vi "Lab 4.vi"() -> ()   [LabVIEW 2025]
uses:
  Lab 4/Control ENUM.ctl
  Lab 3/Control og.ctl
  Lab 3/Control Runners.ctl
  Lab 3/Control Raw.ctl
  <vilib>/Analysis/baseanly.llb/Mean (DBL).vi
  <vilib>/Analysis/NI_AALBase.lvlib
panel:
  in  "File Path":path
  out "HEART RATE ZONES":string[][](array[string])
  out "BPM":cluster{"Time":timestamp[], "Bpm":i32[]}(graph)
  out "XY Graph":T1(graph)
  in  "Stop":bool
  in  "Save":bool
  in  "New":bool
  out "error out":errorcluster
  in  "error in":errorcluster
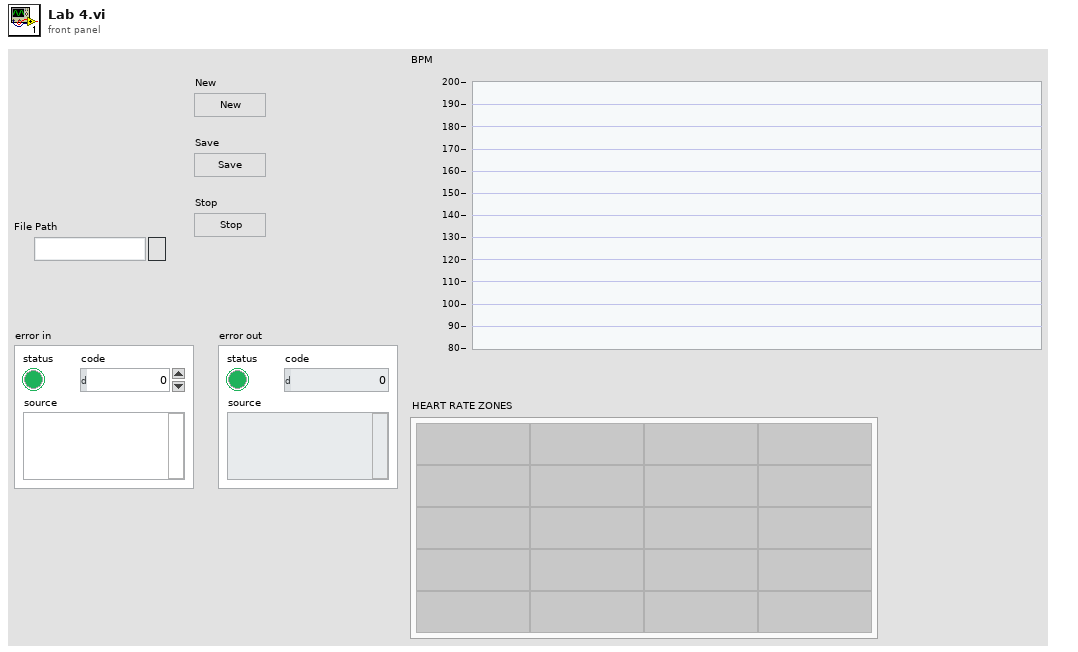
[diagram p1: front panel]
types:
  T1 = cluster{"Total Time in Zone":dbl[], "Heart Rate Zone No":dbl[]}
  T2 = typedef "Control og.ctl" = cluster{"Runner's Data":T3, "HR Max":i32, "Raw Data":T4, "% HR MAX ":dbl[], "HR Zones":string[][], "Heart Rate Zone No":dbl[], "Total Time in Zone":dbl[]}
  T3 = typedef "Control Runners.ctl" = cluster{"Name":string, "Age":i32}
  T4 = typedef "Control Raw.ctl" = cluster{"Time":timestamp[], "Bpm":i32[]}
  T5 = typedef "Control ENUM.ctl" = enum16{"Application Error", "Init", "Idle", "Analyse New Training", "Save", "Error Handling", "Stop"}
  T6 = enum16{"open", "replace", "create", "open or create", "replace or create", "replace or create with confirmation"}
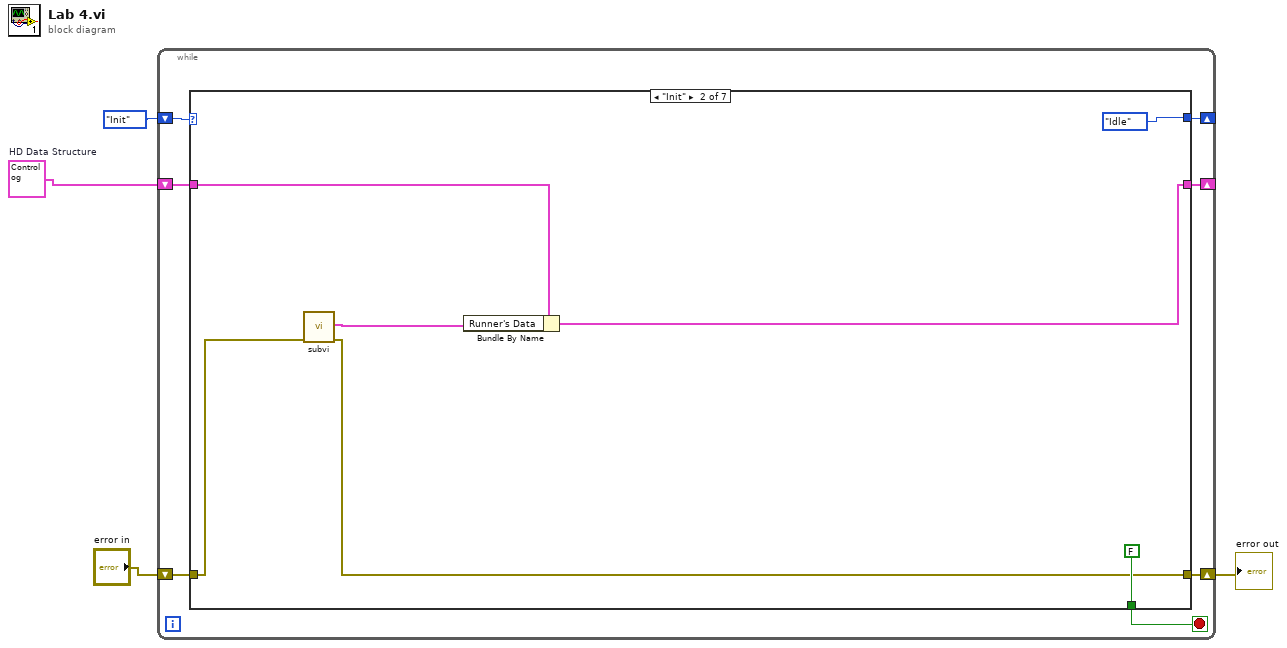
[diagram p0: block diagram]
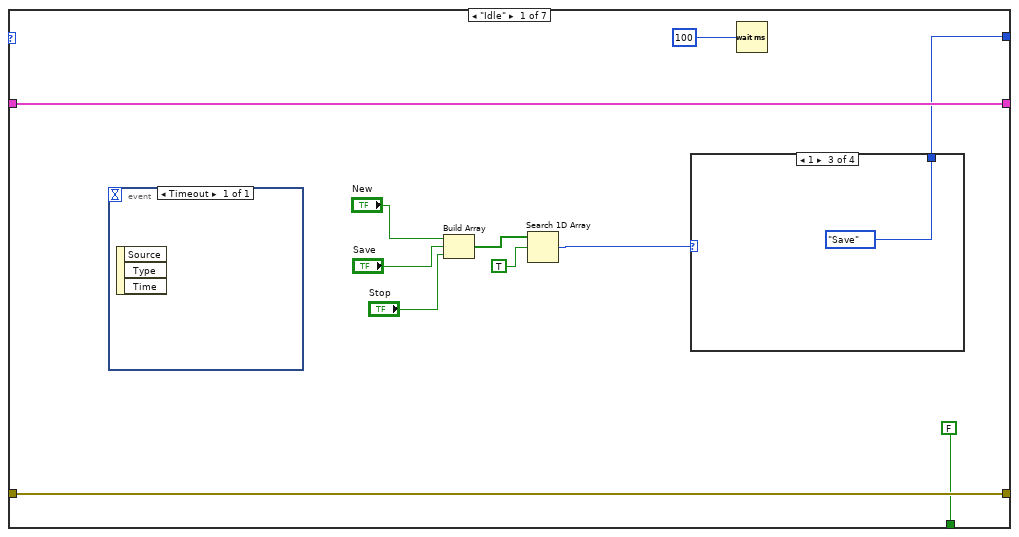
[diagram p2: hidden frame]
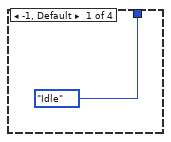
[diagram p3: hidden frame]
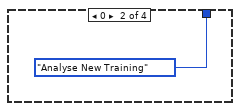
[diagram p4: hidden frame]
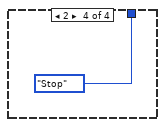
[diagram p5: hidden frame]
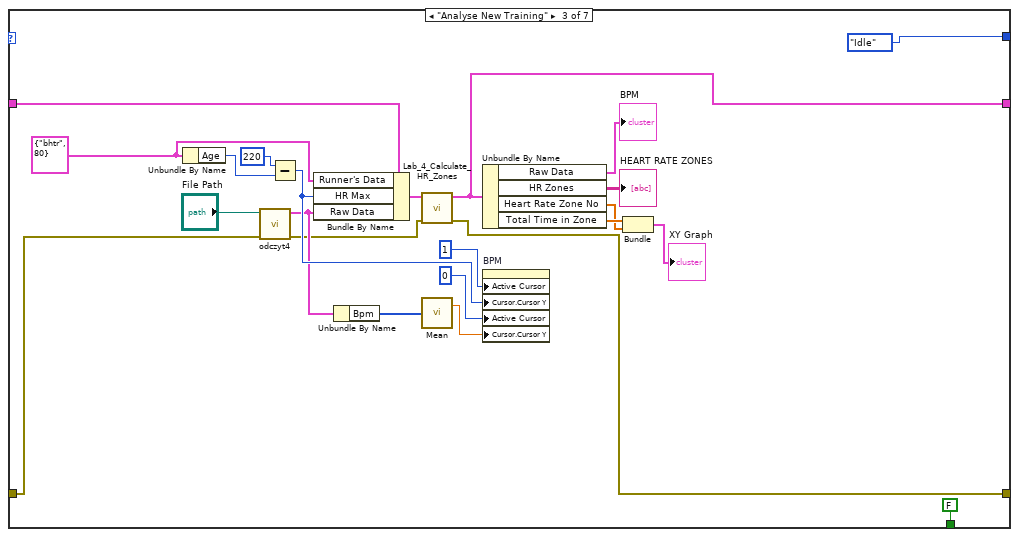
[diagram p6: hidden frame]
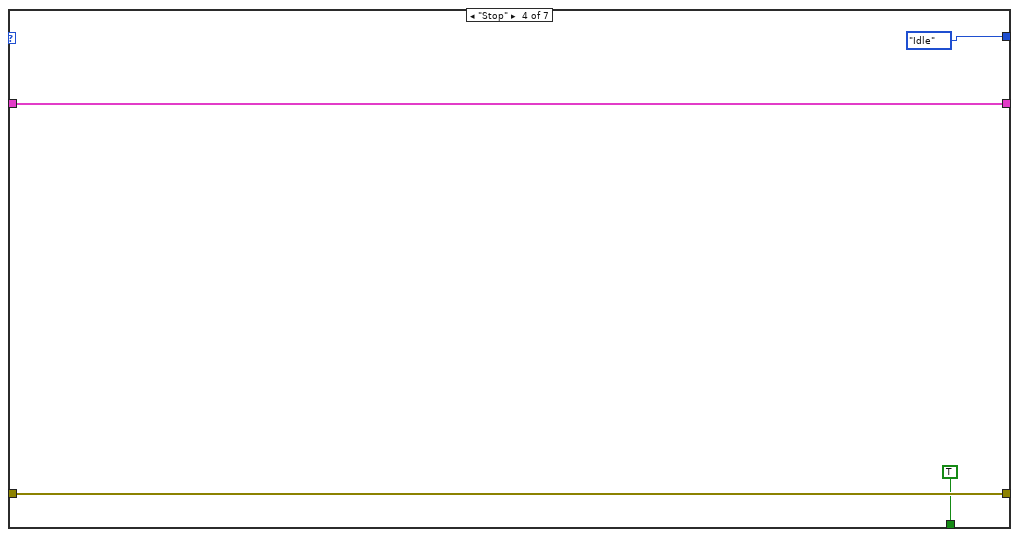
[diagram p7: hidden frame]
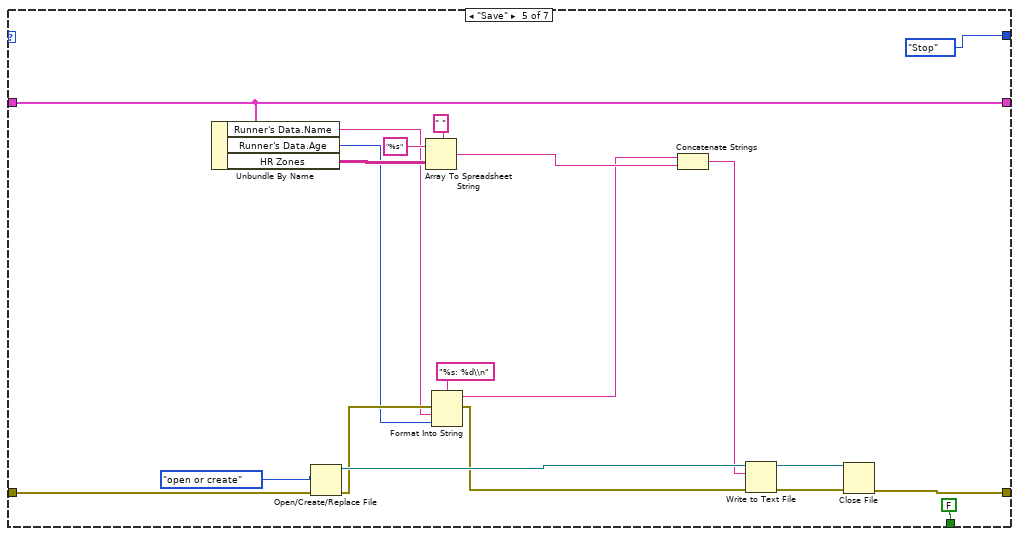
[diagram p8: hidden frame]
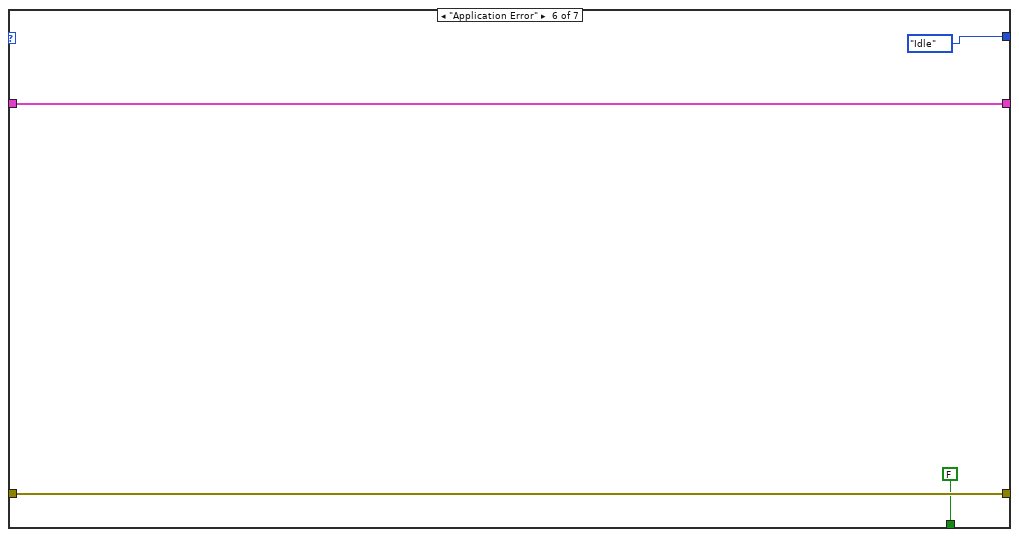
[diagram p9: hidden frame]
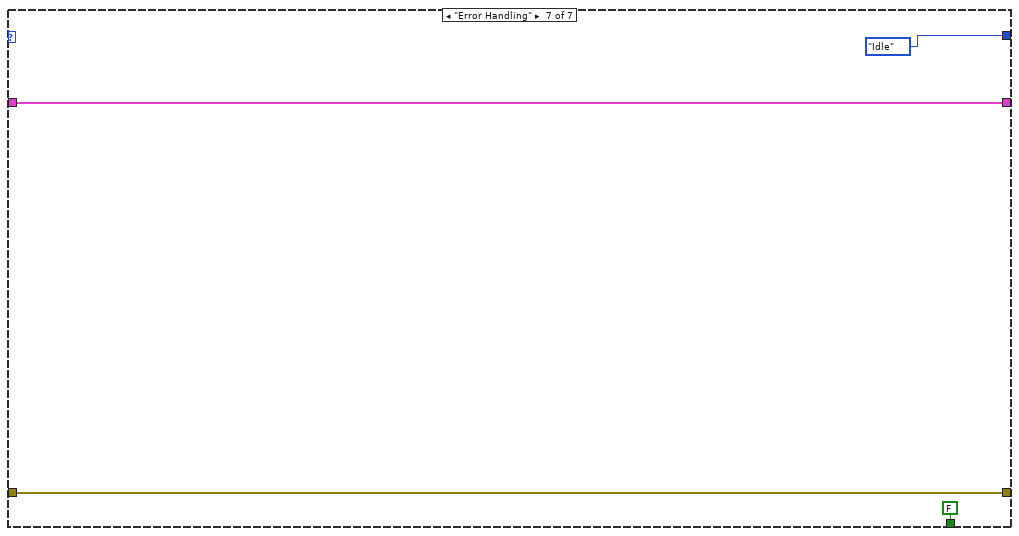
[diagram p10: hidden frame]
diagram:
  w1 = T2 data[18182B]  # HD Data Structure
  n1 = while {
    shift-right: [w11] -> _
    shift-left: w1 -> [w10]
    shift-right: [w8] -> _
    shift-left: Control_ENUM."Init" -> [w9]
    shift-right: [w7] -> w2
    shift-left: "error in" -> [w6]
    stop <- w5 stop-if-true
    n2 = case shown="\"Init\"" w9 {
      tunnel: [w22 w27 w34 w59 w74 w84 w86] -> w11
      tunnel: w10 -> [w22 w28 w37 w59 w74 w84 w86]
      tunnel: [w13 Control_ENUM."Idle" Control_ENUM."Idle" Control_ENUM."Idle" Control_ENUM."Stop" Control_ENUM."Idle" Control_ENUM."Idle"] -> w8
      tunnel: [w21 w30 w42 w58 w78 w83 w88] -> w7
      tunnel: w6 -> [w21 w31 w39 w58 w77 w83 w88]
      tunnel: [FALSE FALSE FALSE TRUE FALSE FALSE FALSE] -> w5
      frame "Idle" {
        n3 = event shown="[0] Timeout" {
          selector: _ -> [_]
          dyn-events: _ -> [_]
          timeout: _ -> [_]
          event Timeout {
            n4 = event-data() -> ()  [unwired: 1 in, 3 out]
          }
        }
        n5 = Build Array("New", "Save", "Stop") -> (w16:bool[])
        n6 = Search 1D Array(1D array=w16, element=TRUE) -> (index of element=w15:i32)  [unwired: 1 in]
        n7 = case shown="1" w15 {
          tunnel: [Control_ENUM."Idle" Control_ENUM."Analyse New Training" Control_ENUM."Save" Control_ENUM."Stop"] -> w13
          frame -1, Default {
          }
          frame 0 {
          }
          frame 1 {
          }
          frame 2 {
          }
        }
        n8 = Wait (ms)(milliseconds to wait=u32 100) -> ()  [unwired: 1 out]
      }
      frame "Init" {
        n9 = call "subvi.vi"("error in"=w31) -> ("error out"=w30:errorcluster, "Runner's Data Ind"=w29:T3)  [unwired: 9 in]
        n10 = Bundle By Name(cluster=w28, "Runner's Data"=w29) -> (w27:T2)
      }
      frame "Analyse New Training" {
        w36 = T3 {"Name"="bhtr", "Age"=80} ("Runner's Data")
        n11 = Unbundle By Name(w36) -> ("Age"=w47:i32)
        n12 = call "odczyt4.vi"("error in"=w39, "Path"="File Path") -> ("error out"=w38:errorcluster, "Raw Data"=w40:T4)  [unwired: 8 in]
        n13 = Subtract(x=220, y=w47) -> (x-y=w53:i32)
        n14 = Bundle By Name(cluster=w37, "Runner's Data"=w36, "HR Max"=w53, "Raw Data"=w40) -> (w43:T2)
        n15 = Unbundle By Name(w40) -> ("Bpm"=w54:i32[])
        n16 = call "Lab_4_Calculate_HR_Zones.vi"("error in"=w38, "HD Data Structure"=w43) -> ("error out"=w42:errorcluster, "HD Data Structure 2"=w34:T2)  [unwired: 8 in]
        n17 = call-poly <vilib>:"Mean.vi"("X"=w54) -> ("mean"=w55:dbl)  [unwired: 1 out]
        n18 = Unbundle By Name(w34) -> ("Raw Data"=→"BPM":T4, "HR Zones"=→"HEART RATE ZONES":string[][], "Heart Rate Zone No"=w50:dbl[], "Total Time in Zone"=w51:dbl[])
        n19 = property on="BPM" class="XYGraph (strict)"("Active Cursor"=u32 1, "Cursor.Cursor Y"=w53, "Active Cursor"=u32 0, "Cursor.Cursor Y"=w55) -> ()  [unwired: 2 in, 2 out]
        n20 = Bundle("Total Time in Zone"=w51, "Heart Rate Zone No"=w50) -> (→"XY Graph":T1)  [unwired: 1 in]
      }
      frame "Stop" {
      }
      frame "Save" {
        n21 = Unbundle By Name(w74) -> ("Runner's Data.Name"=w68:string, "Runner's Data.Age"=w69:i32, "HR Zones"=w73:string[][])
        n22 = Open/Create/Replace File(error in=w77, operation (0:open)=T6."open or create") -> (refnum out=w80:refnum<file>, error out=w70:errorcluster)  [unwired: 4 in, 1 out]
        n23 = Array To Spreadsheet String(delimiter (Tab)=" ", array=w73, 3:"%s" ("format string")) -> (spreadsheet string=w71:string)
        n24 = Format Into String(format string="%s: %d\\n", error in=w70, w68, w69) -> (resulting string=w66:string, error out=w63:errorcluster)  [unwired: 1 in]
        n25 = Concatenate Strings(w66, w71) -> (w65:string)
        n26 = Write to Text File(file (use dialog)=w80, text=w65, error in=w63) -> (refnum out=w79:refnum<file>, error out=w62:errorcluster)  [unwired: 1 in, 1 out]
        n27 = Close File(refnum=w79, error in=w62) -> (error out=w78:errorcluster)  [unwired: 1 out]
      }
      frame "Application Error" {
      }
      frame "Error Handling" {
      }
    }
  }
  "error out" <- w2
